vi "Aufzeichnung_Schritt.vi"(9 "Previous":cluster{"text":string, "count":i32}, 10 "Row":dbl[](array[numeric])=[0.0], 11 "Settings":T1={"record"=FALSE, "clear"=FALSE, "limit"=10000, "header"="", "source"=""}) -> (2 "Full":bool, 3 "Current":cluster{"text":string, "count":i32})   [LabVIEW 2026]
doc: "Append a raw sample only when requested. Bounded memory, source label on every row, no computed laboratory results."
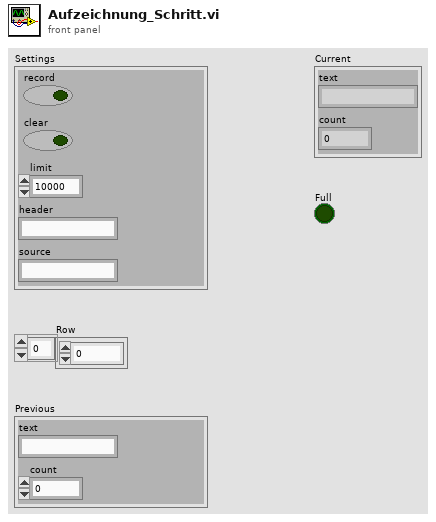
[diagram p1: front panel]
types:
  T1 = cluster{"record":bool, "clear":bool, "limit":i32, "header":string, "source":string}
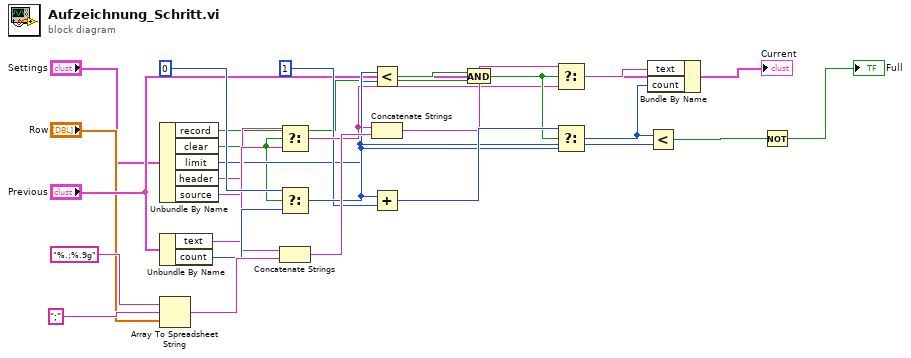
[diagram p0: block diagram]
diagram:
  n1 = Unbundle By Name("Settings") -> ("record"=w4:bool, "clear"=w5:bool, "limit"=w6:i32, "header"=w7:string, "source"=w8:string)
  n2 = Unbundle By Name("Previous") -> ("text"=w9:string, "count"=w10:i32)
  n3 = Array To Spreadsheet String(delimiter (Tab)=";", array="Row", 3:"%.;%.9g") -> (spreadsheet string=w19:string)
  n4 = Select(t=w7, s=w5, f=w9) -> (s? t:f=w13:string)
  n5 = Select(t=0, s=w5, f=w10) -> (s? t:f=w14:i32)
  n6 = Concatenate Strings(w8, w19) -> (w20:string)
  n7 = Less?(x=w14, y=w6) -> (x < y?=w15:bool)
  n8 = Concatenate Strings(w13, w20) -> (w21:string)
  n9 = Add(x=w14, y=1) -> (x+y=w22:i32)
  n10 = And(x=w15, y=w4) -> (x .and. y?=w16:bool)
  n11 = Select(t=w21, s=w16, f=w13) -> (s? t:f=w23:string)
  n12 = Select(t=w22, s=w16, f=w14) -> (s? t:f=w24:i32)
  n13 = Bundle By Name(cluster="Previous", "text"=w23, "count"=w24) -> (→"Current":cluster{"text":string, "count":i32})
  n14 = Less?(x=w24, y=w6) -> (x < y?=w26:bool)
  n15 = Not(x=w26) -> (.not. x?=→"Full":bool)
